vi "MQTT Connect - Post Connect Reconnect.vi"(0 "MQTT Session":T1, 5 "Clean Start":bool, 7 "Session present":bool, 11 "error in":errorcluster) -> (4 "MQTT Session out":T1, 15 "error out":errorcluster)   [LabVIEW 2019, in "KoRE-MQTT.lvlib"]
doc: "Copyright (c) 2026 KoRElibs.com\nSPDX-License-Identifier: EUPL-1.2\n\nThis VI is licensed under the European Union Public License (EUPL) Version 1.2. You may use this VI unmodified in proprietary works. If you distribute a modified version of this file, the modified file must be released under the EUPL-1.2. Full license: https://joinup.ec.europa.eu/asset/eupl/eupl/1.2/\n\nCopyright (c) 2025 KoRElibs.com\nSPDX-License-Identifier: EUPL-1.2\n\nThis VI is licensed under the European Union Public License (EUPL) Version 1.2. You may use this VI unmodified in proprietary works. If you distribute a modified version of this file, the modified file must be released under the EUPL-1.2. Full license: https://joinup.ec.europa.eu/asset/eupl/eupl/1.2/"
uses:
  KoRE-MQTT.lvlib
  Public/TypeDefs/MQTT Client Session.ctl
  TypeDefs/MQTT Subscription - Info.ctl
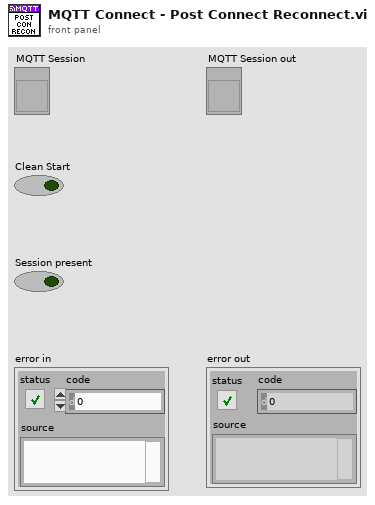
[diagram p1: front panel]
types:
  T1 = typedef "KoRE-MQTT.lvlib/MQTT Client Session.ctl" = refnum<vi>
  T2 = typedef "KoRE-MQTT.lvlib/MQTT Subscription - Info.ctl" = cluster{"Packet Id":u16, "Index":u16, "Identifier":u32, "QoS":u8, "Topic Filter":string, "Reason Code":u8, "Reason String":string, "Granted":bool}
  T3 = typedef "KoRE-MQTT.lvlib/MQTT Client Session - Data.ctl" = cluster{"TCP ref":refnum<k5>, "Next Packet Id":u16, "Version":u8, "Host":string, "Port":u16, "Ping Delta":u32, "Username":string, "Password":string, "Will QoS":u8, "Will Retain":bool, "Will Topic":string, "Will Payload":string, "TCP Timeout":i32, "Semaphore":T4, "In-Flight Messages":variant, "Close":bool, "Last Send":u32, "Keep Alive":u16, "Last Ping RTT":u32, "Last Ping":u32, "Will Properties":T5[], "Session Expiry Interval":u32, "Maximum QoS":u8, "Retain Available":bool, "Server Maximum Packet Size":u32, "Client Identifier":string, "Server Topic Alias Maximum":u16, "Wildcard Subscription Available":bool, "Subscription Identifier Available":bool, "Shared Subscription Available":bool, "Connect Properties":T6[], "Client Maximum Packet Size":u32, "Client Topic Alias Maximum":u16, "Server Receive Maximum":u16, "Client Receive Maximum":u16, "TLS cfg":refnum<k36>, "Subscriptions":T2[]}
  T4 = typedef "Semaphore RefNum" = refnum<k1>
  T5 = typedef "KoRE-MQTT.lvlib/MQTT Property - Will.ctl" = cluster{"Property":u8, "Value":string}
  T6 = typedef "KoRE-MQTT.lvlib/MQTT Property - CONNECT.ctl" = cluster{"Property":u8, "Value":string}
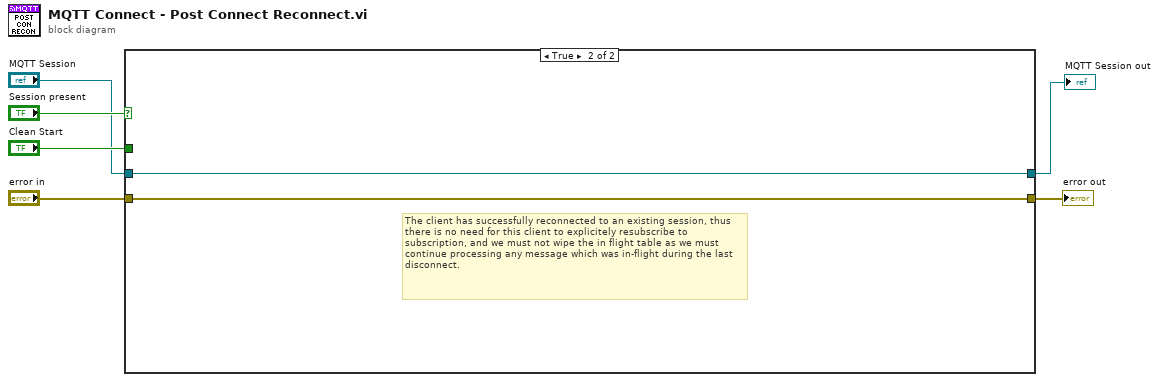
[diagram p0: block diagram]
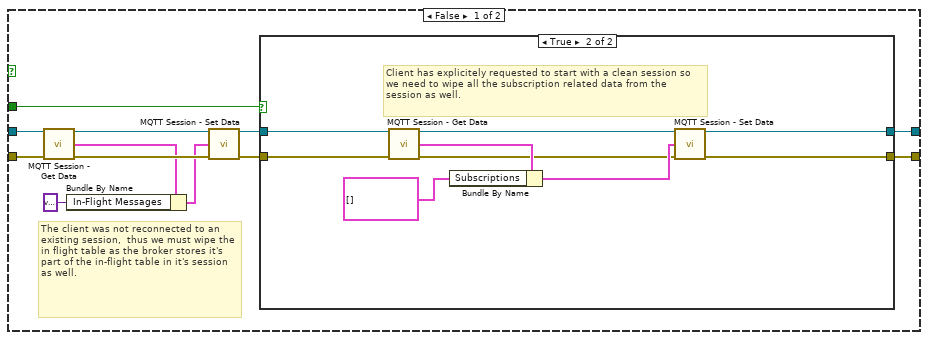
[diagram p2: hidden frame]
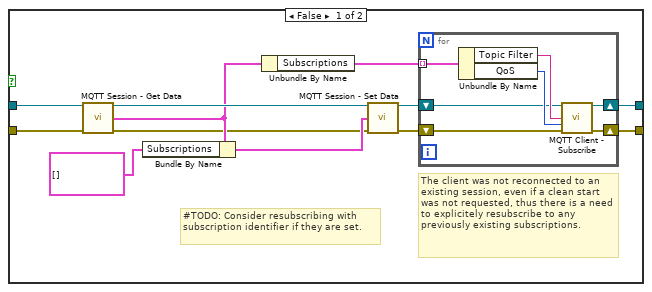
[diagram p3: hidden frame]
diagram:
  n1 = case shown="True" "Session present" {
    tunnel: "MQTT Session" -> [w15 w47]
    tunnel: "Clean Start" -> [w17 _]
    tunnel: "error in" -> [w16 w48]
    tunnel: [w18 w48] -> w2
    tunnel: [w7 w47] -> w1
    frame False {
      # "The client was not reconnected to an existing session,  thus we must wipe the in flight table as the broker stores it's part of the in-flight table in it's session as well."
      n2 = call "MQTT Session - Get Data.vi"("mqtt ref in"=w15, "error in"=w16) -> ("mqtt ref out"=w14:T1, "mqtt ref data"=w10:T3, "error out"=w12:errorcluster)  [unwired: 11 in]
      n3 = Bundle By Name(cluster=w10, "In-Flight Messages"=variant) -> (w9:T3)
      n4 = call "MQTT Session - Set Data.vi"("mqtt ref in"=w14, "mqtt ref data"=w9, "error in"=w12) -> ("mqtt ref out"=w13:T1, "error out"=w11:errorcluster)  [unwired: 11 in]
      n5 = case shown="True" w17 {
        tunnel: w13 -> [w30 w43]
        tunnel: w11 -> [w21 w42]
        tunnel: [w20 w39] -> w18
        tunnel: [w19 w40] -> w7
        frame False {
          # "The client was not reconnected to an existing session, even if a clean start was not requested, thus there is a need to explicitely resubscribe to any previously existing subscriptions."
          # "#TODO: Consider resubscribing with subscription identifier if they are set."
          n6 = call "MQTT Session - Get Data.vi"("mqtt ref in"=w30, "error in"=w21) -> ("mqtt ref out"=w29:T1, "mqtt ref data"=w26:T3, "error out"=w25:errorcluster)  [unwired: 11 in]
          n7 = Bundle By Name(cluster=w26, "Subscriptions"=T2[] []) -> (w28:T3)
          n8 = Unbundle By Name(w26) -> ("Subscriptions"=w24:T2[])
          n9 = call "MQTT Session - Set Data.vi"("mqtt ref in"=w29, "mqtt ref data"=w28, "error in"=w25) -> ("mqtt ref out"=w22:T1, "error out"=w23:errorcluster)  [unwired: 11 in]
          n10 = for {
            tunnel: w24 -> [w37] mode=indexing
            shift-right: [w33] -> w20
            shift-left: w23 -> [w34]
            shift-right: [w31] -> w19
            shift-left: w22 -> [w32]
            n11 = Unbundle By Name(w37) -> ("Topic Filter"=w35:string, "QoS"=w36:u8)
            n12 = call "MQTT Client - Subscribe.vi"("MQTT Session"=w32, "Single Topic Filter"=w35, "Single Topic QoS"=w36, "error in (no error)"=w34) -> ("MQTT Session out"=w31:T1, "error out"=w33:errorcluster)  [unwired: 10 in]
          }
        }
        frame True {
          # "Client has explicitely requested to start with a clean session so we need to wipe all the subscription related data from the session as well."
          n13 = call "MQTT Session - Get Data.vi"("mqtt ref in"=w43, "error in"=w42) -> ("mqtt ref out"=w41:T1, "mqtt ref data"=w45:T3, "error out"=w44:errorcluster)  [unwired: 11 in]
          n14 = Bundle By Name(cluster=w45, "Subscriptions"=T2[] []) -> (w46:T3)
          n15 = call "MQTT Session - Set Data.vi"("mqtt ref in"=w41, "mqtt ref data"=w46, "error in"=w44) -> ("mqtt ref out"=w40:T1, "error out"=w39:errorcluster)  [unwired: 11 in]
        }
      }
    }
    frame True {
      # "The client has successfully reconnected to an existing session, thus there is no need for this client to explicitely resubscribe to subscription, and we must not wipe the in flight table as we must continue processing any message which was in-flight during the last disconnect."
    }
  }
  "error out" <- w2
  "MQTT Session out" <- w1
